vi "Step_IO_Check_Engine.vi"(5 "Target Displacement SP (mm)":dbl=2.5, 6 "Target Flow SP (L/min)":dbl=45.0, 7 "Tolerance (bar)":dbl=2.0, 8 "error in (no error)":errorcluster={"status"=FALSE, "code"=0, "source"="\"\""}, 9 "Target Pressure SP (bar)":dbl=100.0, 10 "Step Name":string="Pressure Step", 11 "Step No":i32=1) -> (0 "error out":errorcluster, 1 "Condition Met":bool, 2 "Actual Power (kW)":dbl, 3 "Actual Flow (L/min)":dbl, 4 "Actual Pressure (bar)":dbl)   [LabVIEW 2026]
doc: "INTENT: Core step I/O check engine. Dispatches setpoints to actuators/plant, interrogates actual sensor feedback, and evaluates condition tolerance."
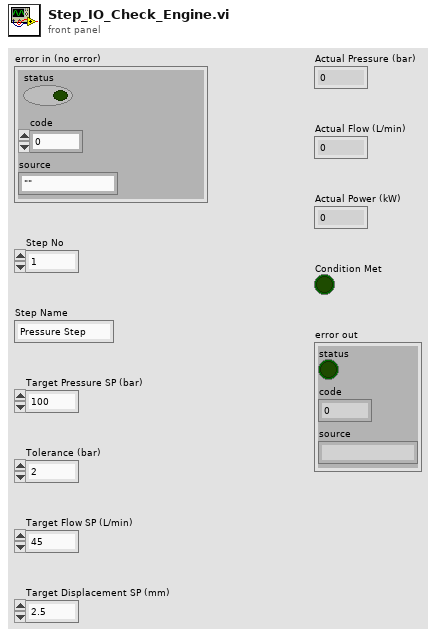
[diagram p1: front panel]
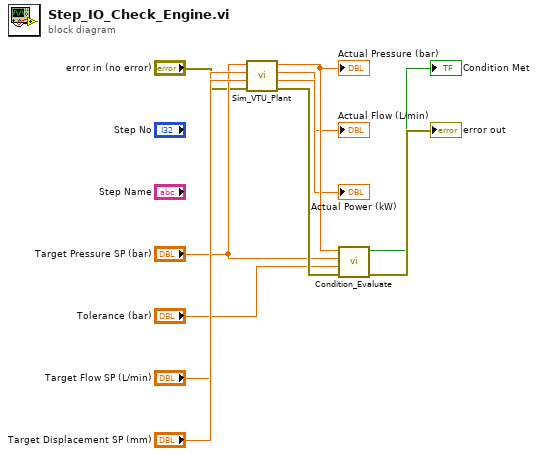
[diagram p0: block diagram]
diagram:
  n1 = call "Sim_VTU_Plant.vi"("error in (no error)"="error in (no error)", "displacement_sp"="Target Displacement SP (mm)", "flow_sp"="Target Flow SP (L/min)", "pressure_sp"="Target Pressure SP (bar)") -> ("error out"=w9:errorcluster, "act_power_kW"=→"Actual Power (kW)":dbl, "act_flow"=→"Actual Flow (L/min)":dbl, "act_pressure"=w8:dbl)  [unwired: 4 in]
  "Actual Pressure (bar)" <- w8
  n2 = call "Condition_Evaluate.vi"("error in (no error)"=w9, "tolerance"="Tolerance (bar)", "target_setpoint"="Target Pressure SP (bar)", "actual_value"=w8) -> ("error out"=→"error out":errorcluster, "condition_met"=→"Condition Met":bool)  [unwired: 6 in]
